vi "set NR Test Channel.vi"(8 "error in (no error)":errorcluster, 9 "Selected CC Argements":T2, 10 "NR Test Channel":T1, 11 "Anritsu Call Box_Implement in":refnum<class "Anritsu Call Box_Implement.lvclass">) -> (0 "error out":errorcluster, 3 "Anritsu Call Box_Implement out":refnum<class "Anritsu Call Box_Implement.lvclass">)   [LabVIEW 2023, in "ANRITSU Call Box.lvlib" / "Anritsu Call Box_Implement.lvclass"]
uses:
  Anritsu Call Box_Implement.lvclass
  Anritsu Call Box_Implement.lvclass/Anritsu Call Box_Implement.ctl
  NR/NR.lvclass
  Type Definition/NR Selected CC Type Arguments.ctl
  ANRITSU Call Box.lvlib
  Type Definition/NR Test Channel Type.ctl
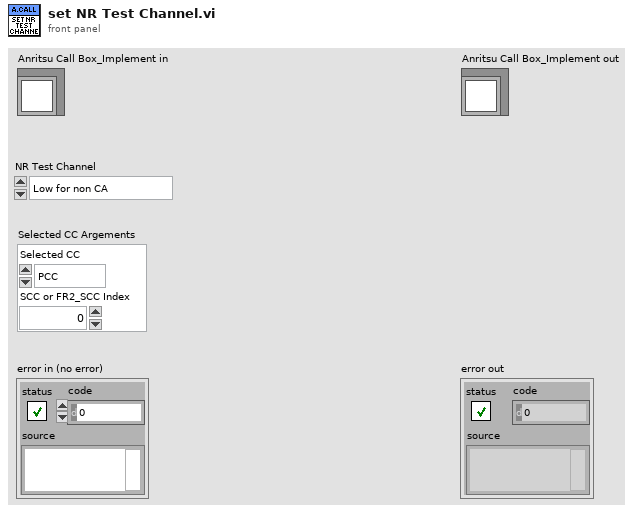
[diagram p1: front panel]
types:
  T1 = typedef "ANRITSU Call Box.lvlib/NR Test Channel Type.ctl" = enum16{"Low for non CA", "Mid for non CA", "High for non CA", "Low for Intra Conti CA", "Mid for Intra Conti CA", "High for Intra Conti CA"}
  T2 = typedef "ANRITSU Call Box.lvlib/NR Selected CC Type Arguments.ctl" = cluster{"Selected CC":enum16{"PCC", "SCC", "FR2_PCC", "FR2_SCC"}, "SCC or FR2_SCC Index":u32}
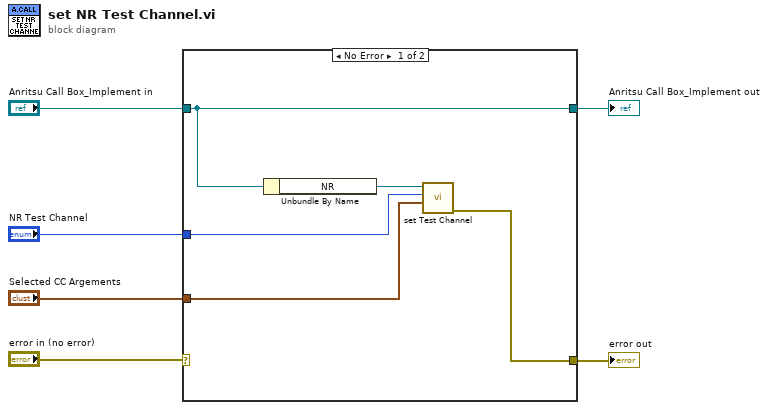
[diagram p0: block diagram]
diagram:
  n1 = case shown="No Error" "error in (no error)" {
    selector: "error in (no error)" -> [_ w12]
    tunnel: "Anritsu Call Box_Implement in" -> [w11 w13]
    tunnel: [w11 w13] -> w5
    tunnel: [w7 w12] -> w3
    tunnel: "Selected CC Argements" -> [w8 _]
    tunnel: "NR Test Channel" -> [w9 _]
    frame No Error {
      n2 = Unbundle By Name(w11) -> ("NR"=w10:refnum<class "NR.lvclass">)
      n3 = call "set Test Channel.vi"("Selected CC Argements"=w8, "NR Test Channel"=w9, "NR in"=w10) -> ("error out"=w7:errorcluster)  [unwired: 7 in, 1 out]
    }
    frame Error {
    }
  }
  "error out" <- w3
  "Anritsu Call Box_Implement out" <- w5
